vi "Connect.vi"(8 "error in (no error)":errorcluster, 10 "Connection String":string, 11 "PostgresqlConnection in":refnum<class "DBC.lvclass">) -> (0 "error out":errorcluster, 3 "PostgresqlConnection out":refnum<class "DBC.lvclass">)   [LabVIEW 2020, in "ORM_pgsql_jdp.lvlib" / "DBC.lvclass"]
uses:
  DBC.lvclass
  C:/Program Files/National Instruments/LabVIEW 2020/vi.lib/Viviota/shared/ORM.lvlibp/DbConnection/DbConnection.lvclass
  <vilib>/JDP Science/PostgreSQL Library/Connection/lib/win32/libpq32.lvclass
  <vilib>/JDP Science/PostgreSQL Library/Connection/lib/win64/libpq64.lvclass
  Write Connection.vi
  <vilib>/Viviota/shared/ORM.lvlibp/DbConnection/Write ColumnNameEqualsValueFormat.vi
  <vilib>/Viviota/shared/ORM.lvlibp/DbConnection/Write ColumnNameFormat.vi
  <vilib>/Viviota/shared/ORM.lvlibp/DbConnection/Write LastIdentityQuery.vi
  <vilib>/Viviota/shared/ORM.lvlibp/DbConnection/Write SupportBulkCreate.vi
  <vilib>/JDP Science/PostgreSQL Library/Connection/PQ Connection.lvclass
panel:
  # "host = hostname\nhostaddr = ipaddress\nport\ndbname\nuser\npassword\nsslmode\nrequiressl (0 or 1)\nconnect_timeout"
  # "host=localhost port=5432 dbname = mydb"
  # "https://www.postgresql.org/docs/17/libpq-connect.html#LIBPQ-PARAMKEYWORDS"
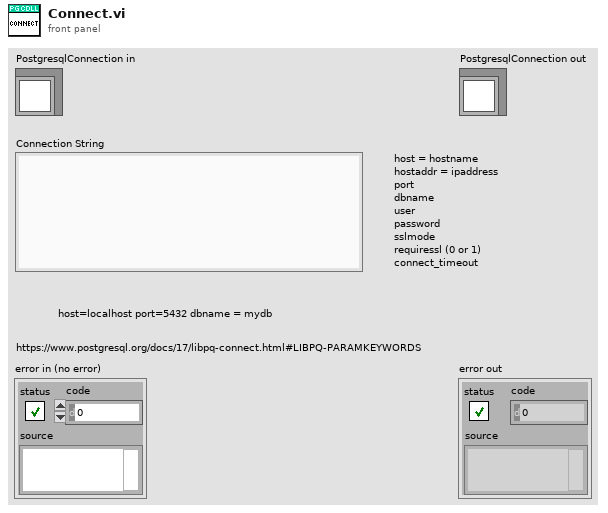
[diagram p1: front panel]
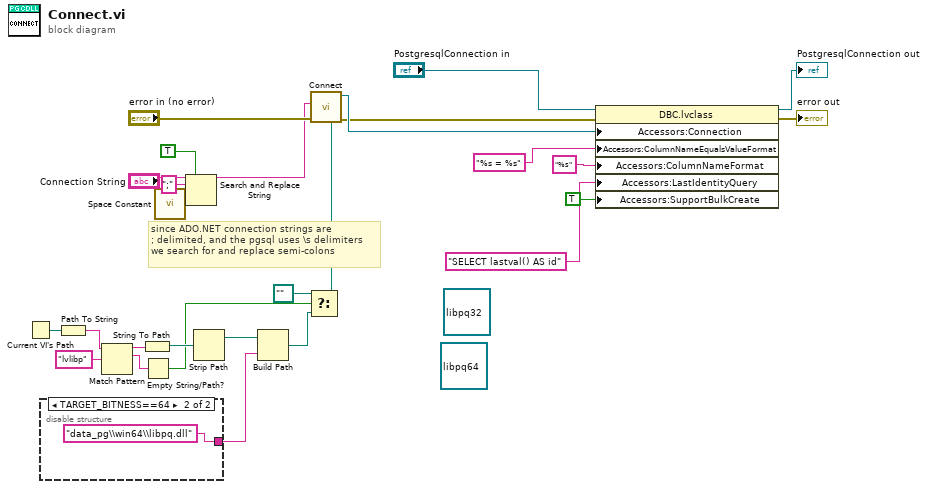
[diagram p0: block diagram]
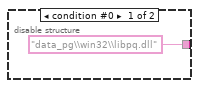
[diagram p2: hidden frame]
diagram:
  (unwired) refnum<class "libpq64.lvclass"> refnum ("PQ Support.lvlib:libpq64.lvclass")
  (unwired) refnum<class "libpq32.lvclass"> refnum ("PQ Support.lvlib:libpq32.lvclass")
  # "since ADO.NET connection strings are\n; delimited, and the pgsql uses \\s delimiters\nwe search for and replace semi-colons"
  n1 = Current VI's Path() -> (path=w12:path)
  n2 = disable-structure shown="TARGET_BITNESS==64" {
    disable-tunnel: ["data_pg\\win32\\libpq.dll" ("regular expression") "data_pg\\win64\\libpq.dll" ("regular expression")] -> w5
    frame condition #0 {
    }
    frame condition #1 (active) {
    }
  }
  n3 = Path To String(path=w12) -> (string=w11:string)
  n4 = Match Pattern(string=w11, regular expression="lvlibp") -> (before substring=w9:string, match substring=w8:string)  [unwired: 1 in, 2 out]
  n5 = String To Path(string=w9) -> (path=w7:path)
  n6 = Empty String/Path?(string/path=w8) -> (empty?=w4:bool)
  n7 = call <vilib>:"Space Constant.vi"() -> ("String"=w17:string)
  n8 = Search and Replace String(replace all?=TRUE ("replace all? (F)"), input string="Connection String", search string=";", replace string=w17) -> (result string=w13:string)  [unwired: 4 in, 3 out]
  n9 = Strip Path(path=w7) -> (stripped path=w6:path)  [unwired: 1 out]
  n10 = Build Path(base path=w6, name or relative path=w5) -> (appended path=w3:path)
  n11 = Select(t=path "", s=w4, f=w3) -> (s? t:f=w1:path)
  n12 = call <vilib>:"Connect.vi"("Override PQ path (optional)"=w1, "error in (no error)"="error in (no error)", "Connection Strings"=w13) -> ("error out"=w14:errorcluster, "PQ Connection"=w15:refnum<class "PQ Connection.lvclass">)  [unwired: 7 in]
  n13 = property class="DBC.lvclass"(reference="PostgresqlConnection in", error in=w14, "Accessors:Connection"=w15, "Accessors:ColumnNameEqualsValueFormat"="%s = %s" ("ColumnNameFormat"), "Accessors:ColumnNameFormat"="%s" ("ColumnNameFormat"), "Accessors:LastIdentityQuery"="SELECT lastval() AS id" ("LastIdentityQuery"), "Accessors:SupportBulkCreate"=TRUE ("SupportBulkCreate")) -> (reference out=→"PostgresqlConnection out":refnum<class "DBC.lvclass">, error out=→"error out":errorcluster)
